vi "calculate_strain__4b50c51ef9.vi"(6 "commanded strain":dbl[](array[numeric]), 7 "real strain":dbl[](array[numeric]), 9 "Gap":dbl, 10 "voltage to displacement contant":dbl, 11 "initial position in volt":dbl) -> (2 "real strain (-)":dbl[](array[numeric]), 3 "commanded strain (-)":dbl[](array[numeric]))   [LabVIEW 2023]
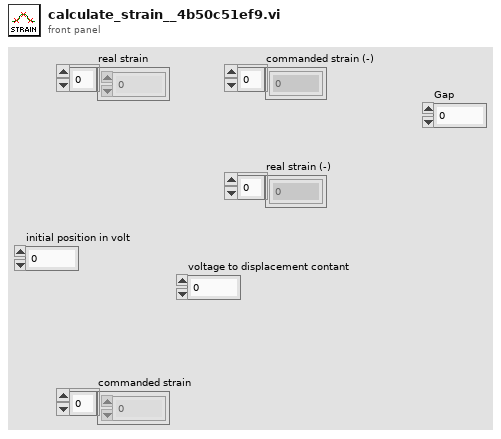
[diagram p1: front panel]
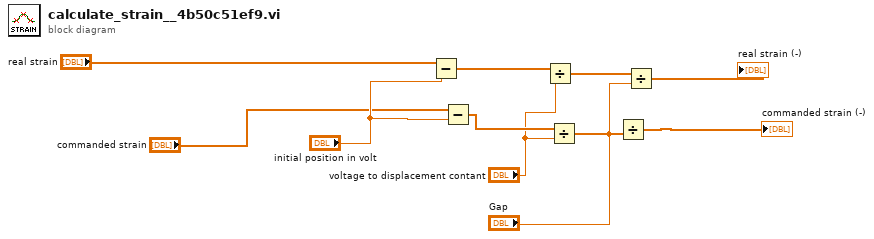
[diagram p0: block diagram]
diagram:
  n1 = Subtract(x="real strain", y="initial position in volt") -> (x-y=w8:dbl[])
  n2 = Subtract(x="commanded strain", y="initial position in volt") -> (x-y=w10:dbl[])
  n3 = Divide(x=w8, y="voltage to displacement contant") -> (x/y=w9:dbl[])
  n4 = Divide(x=w10, y="voltage to displacement contant") -> (x/y=w7:dbl[])
  n5 = Divide(x=w7, y="Gap") -> (x/y=→"commanded strain (-)":dbl[])
  n6 = Divide(x=w9, y="Gap") -> (x/y=→"real strain (-)":dbl[])
